vi "Main.vi"() -> ()   [LabVIEW 2019]
doc: "The myRIO Project template acquires acceleration data from the onboard accelerometer and displays the changes of acceleration values in a waveform chart."
panel:
  in  "Stop Button":bool
  in  "盆數(計時端)":i32
  in  "盆數(電腦端)":i32
  out "error out":errorcluster
  in  "目標(計時端)":i32
  in  "目標(電腦端)":i32
  in  "出發(計時端)":bool=TRUE
  in  "出發(電腦端)":bool=TRUE
  in  "開始":bool
  in  "error in (no error)":errorcluster
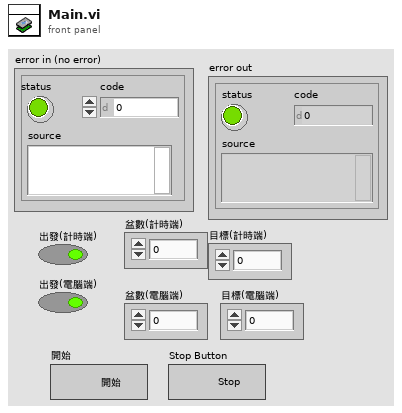
[diagram p1: front panel]
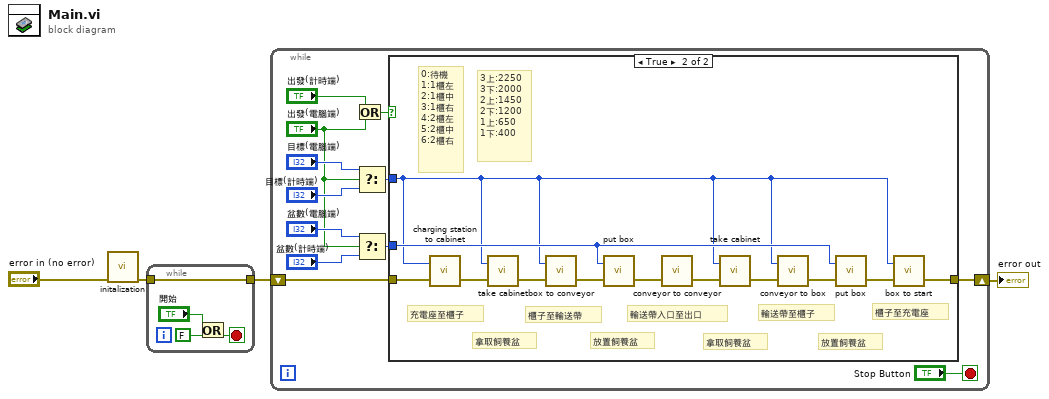
[diagram p0: block diagram]
diagram:
  n1 = call "initalization.vi"("error in (no error)"="error in (no error)") -> ("error out"=w3:errorcluster)  [unwired: 10 in]
  n2 = while {
    tunnel: w3 -> [w5]
    tunnel: [w5] -> w2
    stop <- w8 stop-if-true
    n3 = Or(x="開始", y=FALSE) -> (x .or. y?=w8:bool)
  }
  n4 = while {
    shift-right: [w14] -> w1
    shift-left: w2 -> [w15]
    stop <- "Stop Button" stop-if-true
    n5 = Or(x="出發(計時端)", y="出發(電腦端)") -> (x .or. y?=w19:bool)
    n6 = Select(t="目標(電腦端)", s="出發(電腦端)", f="目標(計時端)") -> (s? t:f=w16:i32)
    n7 = Select(t="盆數(電腦端)", s="出發(電腦端)", f="盆數(計時端)") -> (s? t:f=w10:i32)
    n8 = case shown="True" w19 {
      tunnel: w16 -> [_ w22]
      tunnel: w15 -> [w21 w33]
      tunnel: [w21 w24] -> w14
      tunnel: w10 -> [_ w23]
      frame False {
      }
      frame True {
        # "櫃子至充電座"
        # "放置飼養盆"
        # "輸送帶至櫃子"
        # "拿取飼養盆"
        # "輸送帶入口至出口"
        # "放置飼養盆"
        # "櫃子至輸送帶"
        # "拿取飼養盆"
        # "充電座至櫃子"
        # "3上:2250\n3下:2000\n2上:1450\n2下:1200\n1上:650\n1下:400"
        # "0:待機\n1:1櫃左\n2:1櫃中\n3:1櫃右\n4:2櫃左\n5:2櫃中\n6:2櫃右"
        n9 = call "charging station to cabinet.vi"("error in (no error)"=w33, "目標位置"=w22) -> ("error out"=w32:errorcluster)  [unwired: 1 in]
        n10 = call "take cabinet.vi"("error in (no error)"=w32, "高度"=w22) -> ("error out"=w31:errorcluster)  [unwired: 1 in]
        n11 = call "box to conveyor.vi"("error in (no error)"=w31, "櫃子"=w22) -> ("error out"=w30:errorcluster)  [unwired: 1 in]
        n12 = call "put box.vi"("error in (no error)"=w30, "盆數"=w23) -> ("error out"=w29:errorcluster)  [unwired: 1 in]
        n13 = call "conveyor to conveyor.vi"("error in (no error)"=w29) -> ("error out"=w28:errorcluster)  [unwired: 2 in]
        n14 = call "take cabinet.vi"("error in (no error)"=w28, "高度"=w22) -> ("error out"=w27:errorcluster)  [unwired: 1 in]
        n15 = call "conveyor to box.vi"("error in (no error)"=w27, "櫃子"=w22) -> ("error out"=w26:errorcluster)  [unwired: 1 in]
        n16 = call "put box.vi"("error in (no error)"=w26, "盆數"=w23) -> ("error out"=w25:errorcluster)  [unwired: 1 in]
        n17 = call "box to start.vi"("error in (no error)"=w25, "櫃子"=w22) -> ("error out"=w24:errorcluster)  [unwired: 1 in]
      }
    }
  }
  "error out" <- w1
